vi "Modify Files.vi"() -> ()   [LabVIEW 2015]
uses:
  <vilib>/regexp/Match Regular Expression.xnode
  <userlib>/_OpenG.lib/file/file.llb/Strip Path Extension - String__ogtk.vi
panel:
  out "Array 2":T1(array[cluster])
  out "Array":path[](array[path])
  out "size(s) 2":i32
  out "size(s)":i32
  out "spreadsheet string":string
  # "UFileCrc32"
  # "INPUT: at blockdiagramm"
  # "Look out: some  *.pas files  do  not have a *.dcu file\nwhen included like\n{$I I_Connector_Diff.pas}"
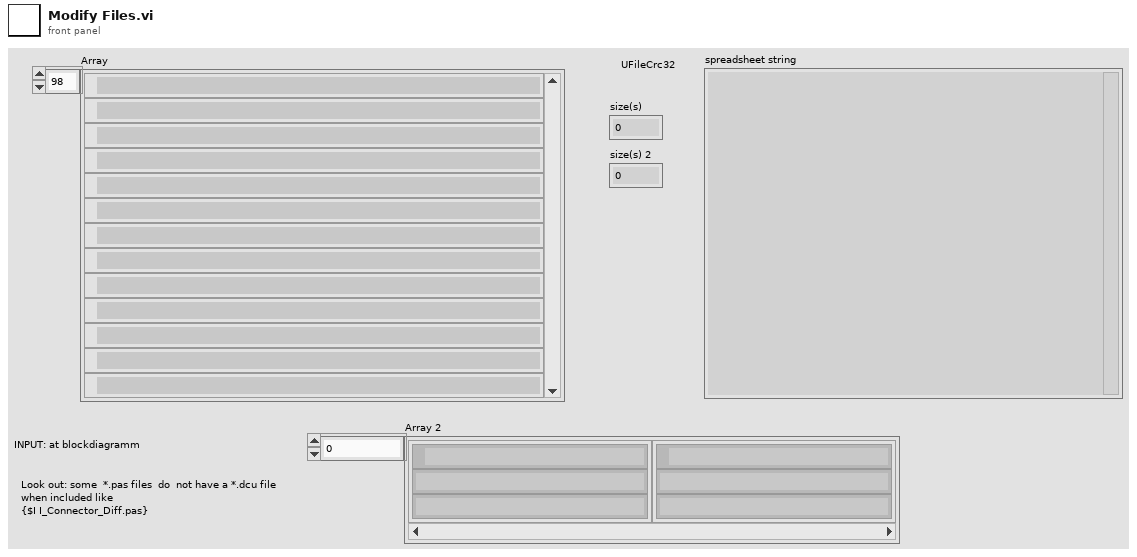
[diagram p1: front panel]
types:
  T1 = cluster{"Path":path, "whole match":string, string}[]
  T2 = enum16{"DebInit add Exit", "Find DebInit", "Find DebFinal", "DebInit with Exit to InitFinal_Add", "uses add InitFinal_List", "add Unit_Name", "InitFinal_Add adapt", "Add InitVars_Dll", "Find Without InitVars_Dll"}
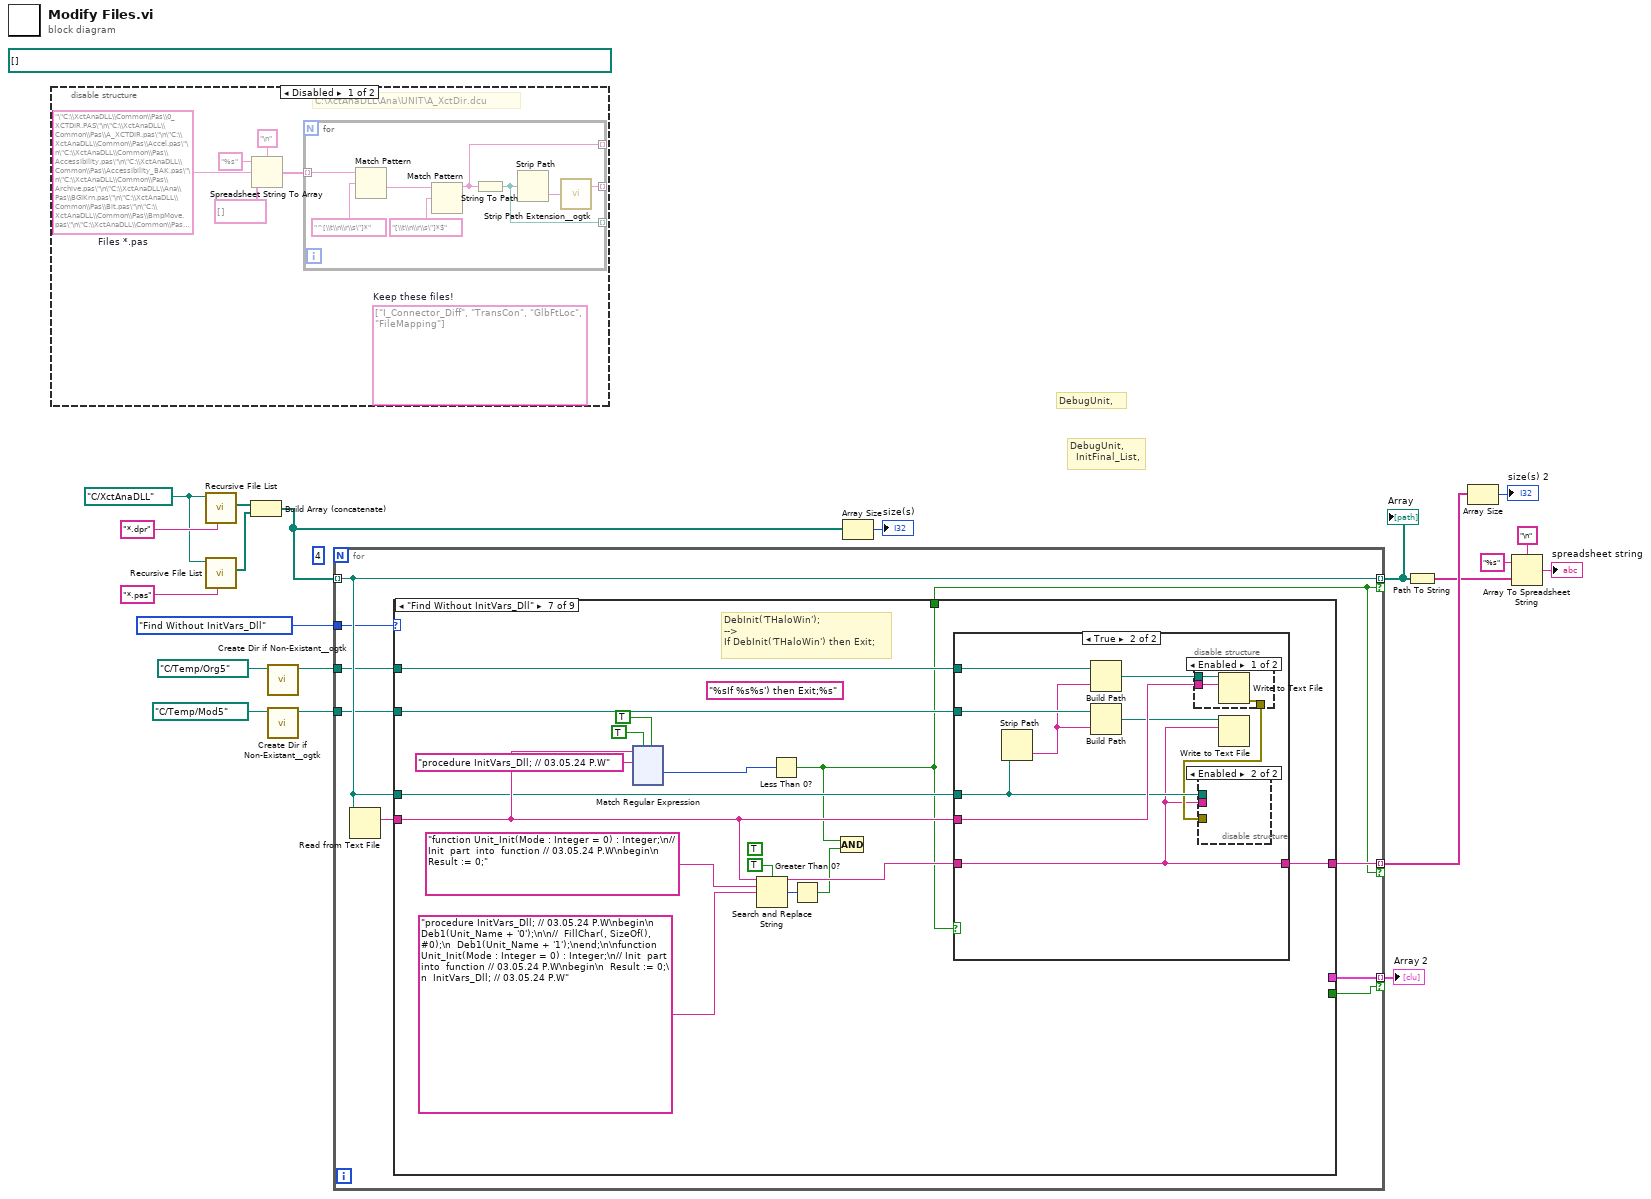
[diagram p0: block diagram]
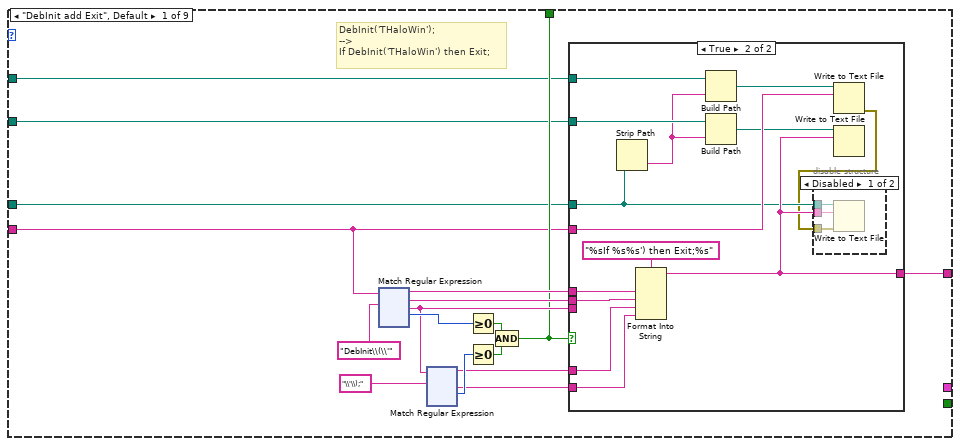
[diagram p3: hidden frame]
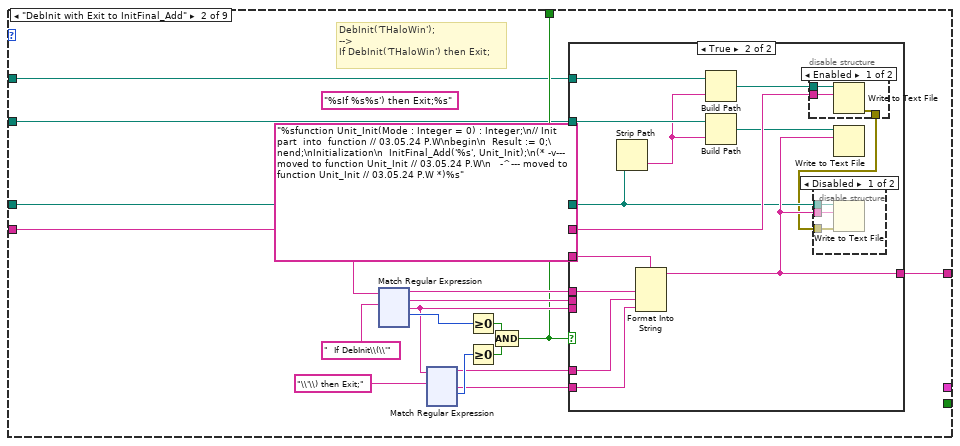
[diagram p6: hidden frame]
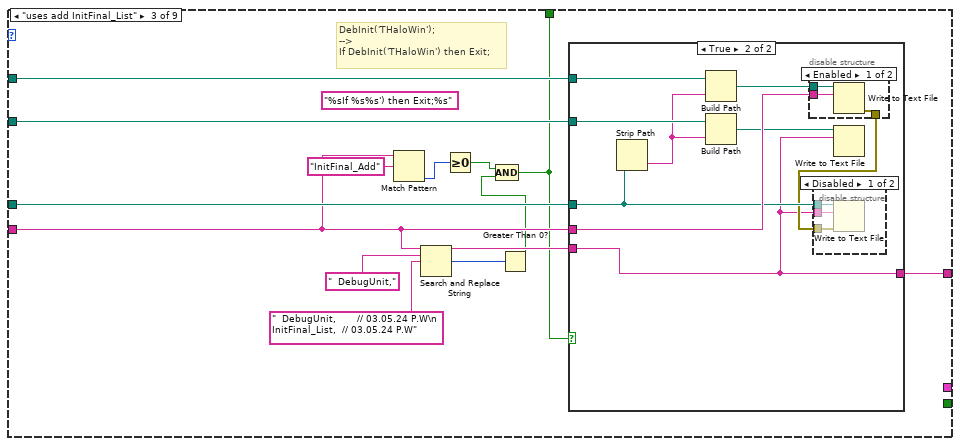
[diagram p10: hidden frame]
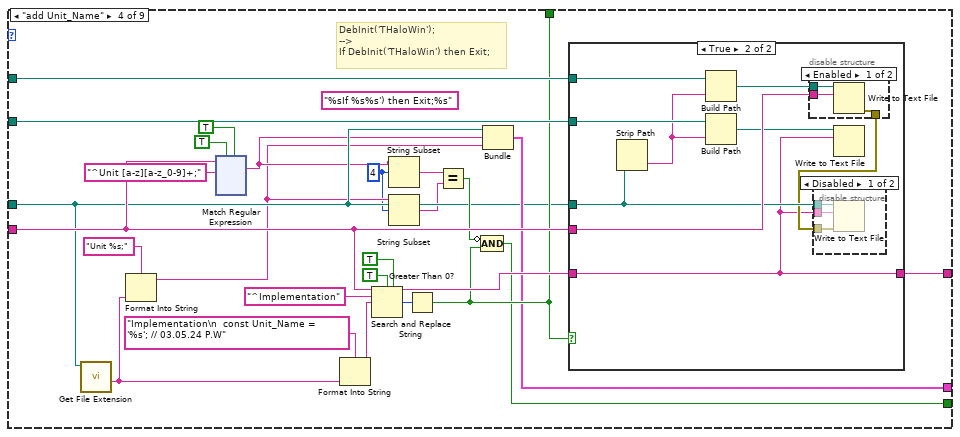
[diagram p14: hidden frame]
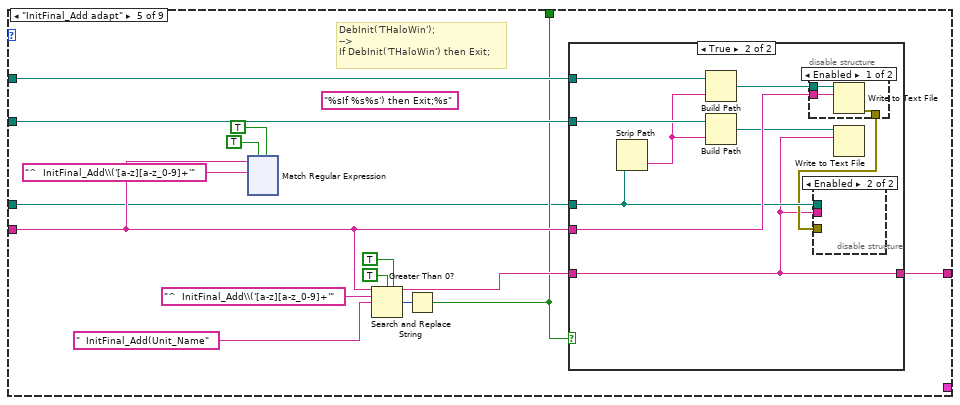
[diagram p18: hidden frame]
diagram:
  (unwired) 4
  w6 = path "C:/XctAnaDLL" ("Folder Path")
  (unwired) path[] []
  # "DebugUnit,\n  InitFinal_List,"
  # "DebugUnit,"
  n1 = disable-structure shown="Disabled" {
    frame Disabled {
      (unwired) string[] ["I_Connector_Diff", "TransCon", "GlbFtLoc", "FileMapping"]  # Keep these files!
      w22 = "\"C:\\XctAnaDLL\\Common\\Pas\\0_XCTDIR.PAS\"\n\"C:\\XctAnaDLL\\Common\\Pas\\A_XCTDIR.pas\"\n\"C:\\XctAnaDLL\\Common\\Pas\\Accel.pas\"\n\"C:\\XctAnaDLL\\Common\\Pas\\Accessibility.pas\"\n\"C:\\XctAnaDLL\\Common\\Pas\\Accessibility_BAK.pas\"\n\"C:\\XctAnaDLL\\Common\\Pas\\Archive.pas\"\n\"C:\\XctAnaDLL\\Ana\\Pas\\BGIKrn.pas\"\n\"C:\\XctAnaDLL\\Common\\Pas\\Bit.pas\"\n\"C:\\XctAnaDLL\\Common\\Pas\\BmpMove.pas\"\n\"C:\\XctAnaDLL\\Common\\Pas\\BmpStack.pas\"\n\"C:\\XctAnaDLL\\Common\\Pas\\BmpUse.pas\"\n\"C:\\XctAnaDLL\\Common\\Pas\\BNHead0.pas\"\n\"C:\\XctAnaDLL\\Ana\\Pas\\BNKEY0.pas\"\n\"C:\\XctAnaDLL\\Ana\\Pas\\BnKnDaKo.pas\"\n\"C:\\XctAnaDLL\\Ana\\Pas\\BNLOCK.pas\"\n\"C:\\XctAnaDLL\\Ana\\Pas\\BufferNumbers.pas\"\n\"C:\\XctAnaDLL\\Ana\\Pas\\BufferNumbers_2.pas\"\n\"C:\\XctAnaDLL\\Ana\\Pas\\Calc.pas\"\n\"C:\\XctAnaDLL\\Common\\Pas\\CheckDat.pas\"\n\"C:\\XctAnaDLL\\Common\\Pas\\CheckPrevious.pas\"\n\"C:\\XctAnaDLL\\Ana\\Pas\\CHK540UP.PAS\"\n\"C:\\XctAnaDLL\\Common\\Pas\\ChkSum.pas\"\n\"C:\\XctAnaDLL\\Ana\\Pas\\ChngSide.pas\"\n\"C:\\XctAnaDLL\\Common\\Pas\\ClientViewXctImagesUnit.pas\"\n\"C:\\XctAnaDLL\\Common\\Pas\\ClipBrdUse.pas\"\n\"C:\\XctAnaDLL\\Ana\\Pas\\cmConst.pas\"\n\"C:\\XctAnaDLL\\Ana\\Pas\\CMDPARAM.PAS\"\n\"C:\\XctAnaDLL\\Common\\Pas\\CodeFind.pas\"\n\"C:\\XctAnaDLL\\Common\\Pas\\ColorDlgUse.pas\"\n\"C:\\XctAnaDLL\\Common\\Pas\\ColorModels.pas\"\n\"C:\\XctAnaDLL\\Common\\Pas\\ColorsPlus.pas\"\n\"C:\\XctAnaDLL\\Info\\TempTest\\COMAC000_Msk.pas\"\n\"C:\\XctAnaDLL\\Info\\TempTest\\COMACFEM_Msk.pas\"\n\"C:\\XctAnaDLL\\Common\\Pas\\ComNames.pas\"\n\"C:\\XctAnaDLL\\Common\\Pas\\ComparePathes.pas\"\n\"C:\\XctAnaDLL\\Common\\Pas\\Complexs.pas\"\n\"C:\\XctAnaDLL\\Ana\\Pas\\CONF.PAS\"\n\"C:\\XctAnaDLL\\Common\\Pas\\ControlsUse.pas\"\n\"C:\\XctAnaDLL\\Common\\Pas\\Crt.pas\"\n\"C:\\XctAnaDLL\\Ana\\Pas\\CSV2PAL.pas\"\n\"C:\\XctAnaDLL\\Ana\\Pas\\csvread.pas\"\n\"C:\\XctAnaDLL\\Ana\\Pas\\CSVSTAT.pas\"\n\"C:\\XctAnaDLL\\Ana\\Pas\\CVDOSTXT.PAS\"\n\"C:\\XctAnaDLL\\Common\\Pas\\DataBaseXct.pas\"\n\"C:\\XctAnaDLL\\Common\\Pas\\DebInit.pas\"\n\"C:\\XctAnaDLL\\Common\\Pas\\DebugForm.pas\"\n\"C:\\XctAnaDLL\\Ana\\Pas\\DefDrvs.pas\"\n\"C:\\XctAnaDLL\\Common\\Pas\\DefHTMLOpts.pas\"\n\"C:\\XctAnaDLL\\Common\\Pas\\DelphiCrt.pas\"\n\"C:\\XctAnaDLL\\Common\\Pas\\DialogsSecure.pas\"\n\"C:\\XctAnaDLL\\Common\\Pas\\DIBTools.pas\"\n\"C:\\XctAnaDLL\\Common\\Pas\\DirTool.pas\"\n\"C:\\XctAnaDLL\\Common\\Pas\\DiskTyp.pas\"\n\"C:\\XctAnaDLL\\Common\\Pas\\DlgDeltaTime.pas\"\n\"C:\\XctAnaDLL\\Ana\\Pas\\Do540up.pas\"\n\"C:\\XctAnaDLL\\Ana\\Pas\\DoModify.pas\"\n\"C:\\XctAnaDLL\\Common\\Pas\\Dos.pas\"\n\"C:\\XctAnaDLL\\Common\\Pas\\DosGlb.pas\"\n\"C:\\XctAnaDLL\\Common\\Pas\\DosTimer.pas\"\n\"C:\\XctAnaDLL\\Common\\Pas\\Draw.pas\"\n\"C:\\XctAnaDLL\\Common\\Pas\\DrawGridDialog.pas\"\n\"C:\\XctAnaDLL\\Ana\\Pas\\DUMMY.PAS\"\n\"C:\\XctAnaDLL\\Common\\Pas\\EE_Param.pas\"\n\"C:\\XctAnaDLL\\Common\\Pas\\EE_Param_RW.pas\"\n\"C:\\XctAnaDLL\\Common\\Pas\\EE_Param_Tools.pas\"\n\"C:\\XctAnaDLL\\Common\\Pas\\ErrConst.pas\"\n\"C:\\XctAnaDLL\\Common\\Pas\\EventLog.pas\"\n\"C:\\XctAnaDLL\\Common\\Pas\\EventLogs.pas\"\n\"C:\\XctAnaDLL\\Ana\\Pas\\ExGraph.pas\"\n\"C:\\XctAnaDLL\\Common\\Pas\\ExitTool.pas\"\n\"C:\\XctAnaDLL\\Ana\\Pas\\EXTPLUS.pas\"\n\"C:\\XctAnaDLL\\Ana\\Pas\\FCOUNT.pas\"\n\"C:\\XctAnaDLL\\Common\\Pas\\FemGlb.pas\"\n\"C:\\XctAnaDLL\\Common\\Pas\\FemurPcForm1.pas\"\n\"C:\\XctAnaDLL\\Common\\Pas\\FFTs.pas\"\n\"C:\\XctAnaDLL\\Delphi\\FileMapping.pas\"\n\"C:\\XctAnaDLL\\Common\\Pas\\FileUtils.pas\"\n\"C:\\XctAnaDLL\\Ana\\Pas\\FindEdge.pas\"\n\"C:\\XctAnaDLL\\Common\\Pas\\FirFilter.pas\"\n\"C:\\XctAnaDLL\\Common\\Pas\\FormatedList.pas\"\n\"C:\\XctAnaDLL\\Common\\Pas\\FormatTools.pas\"\n\"C:\\XctAnaDLL\\Ana\\Pas\\formLoopEdit.pas\"\n\"C:\\XctAnaDLL\\Common\\Pas\\FormMountImage.pas\"\n\"C:\\XctAnaDLL\\Ana\\FormTranslate.pas\"\n\"C:\\XctAnaDLL\\Common\\Pas\\Fourier.pas\"\n\"C:\\XctAnaDLL\\Common\\Pas\\FramePaint.pas\"\n\"C:\\XctAnaDLL\\Common\\Pas\\Frames.pas\"\n\"C:\\XctAnaDLL\\Common\\Pas\\FrameScrolledImage.pas\"\n\"C:\\XctAnaDLL\\Common\\Pas\\FrameScrolledImageTool.pas\"\n\"C:\\XctAnaDLL\\Common\\Pas\\FrameToolRect.pas\"\n\"C:\\XctAnaDLL\\Common\\Pas\\frmBnLockPassWd.pas\"\n\"C:\\XctAnaDLL\\Common\\Pas\\frmHexEdit_U.pas\"\n\"C:\\XctAnaDLL\\Common\\Pas\\frmImage.pas\"\n\"C:\\XctAnaDLL\\Common\\Pas\\frmOptsFilesHyperlink.pas\"\n\"C:\\XctAnaDLL\\Common\\Pas\\FrmXCTAbout.pas\"\n\"C:\\XctAnaDLL\\Common\\Pas\\GdiPlusUse.pas\"\n\"C:\\XctAnaDLL\\Common\\Pas\\GeoTools.pas\"\n\"C:\\XctAnaDLL\\Common\\Pas\\GetMovit.pas\"\n\"C:\\XctAnaDLL\\Common\\Pas\\GetTast.pas\"\n\"C:\\XctAnaDLL\\Common\\Pas\\GIFImage.pas\"\n\"C:\\XctAnaDLL\\Common\\Pas\\Glb.pas\"\n\"C:\\XctAnaDLL\\Common\\Pas\\GlbDecs.pas\"\n\"C:\\XctAnaDLL\\Common\\Pas\\GlbFT.pas\"\n\"C:\\XctAnaDLL\\Ana\\Pas\\GlbFtLoc.Pas\"\n\"C:\\XctAnaDLL\\Common\\Pas\\GlbFtLoc.Pas\"\n\"C:\\XctAnaDLL\\Common\\Pas\\GlbHotKey.pas\"\n\"C:\\XctAnaDLL\\Common\\Pas\\GlbKey.pas\"\n\"C:\\XctAnaDLL\\Common\\Pas\\GlbPath.pas\"\n\"C:\\XctAnaDLL\\Common\\Pas\\Glbtools.pas\"\n\"C:\\XctAnaDLL\\Common\\Pas\\GlbType.pas\"\n\"C:\\XctAnaDLL\\Ana\\Pas\\GoXctDir.pas\"\n\"C:\\XctAnaDLL\\Common\\Pas\\Gr_Crt.pas\"\n\"C:\\XctAnaDLL\\Common\\Pas\\Graph0.pas\"\n\"C:\\XctAnaDLL\\Common\\Pas\\GraphGlb.pas\"\n\"C:\\XctAnaDLL\\Common\\Pas\\GraphicsExt.pas\"\n\"C:\\XctAnaDLL\\Common\\Pas\\GridBasic.pas\"\n\"C:\\XctAnaDLL\\Ana\\Pas\\HelpFile.pas\"\n\"C:\\XctAnaDLL\\Common\\Pas\\I_Connector_Diff.pas\"\n\"C:\\XctAnaDLL\\Common\\Pas\\IfTool.pas\"\n\"C:\\XctAnaDLL\\Common\\Pas\\ImgBuf.pas\"\n\"C:\\XctAnaDLL\\Common\\Pas\\ImgMeasTools.pas\"\n\"C:\\XctAnaDLL\\Common\\Pas\\ImgOverview.pas\"\n\"C:\\XctAnaDLL\\Common\\Pas\\IniFilesUse.pas\"\n\"C:\\XctAnaDLL\\Common\\Pas\\IntChar.pas\"\n\"C:\\XctAnaDLL\\Ana\\Pas\\Intopaz.pas\"\n\"C:\\XctAnaDLL\\Common\\Pas\\IoErr.pas\"\n\"C:\\XctAnaDLL\\Common\\Pas\\IOTools.pas\"\n\"C:\\XctAnaDLL\\Common\\Pas\\JobParameter.pas\"\n\"C:\\XctAnaDLL\\JPEG\\jpeg.pas\"\n\"C:\\XctAnaDLL\\Common\\Pas\\JpgUse.pas\"\n\"C:\\XctAnaDLL\\Common\\Pas\\KeyCodes.pas\"\n\"C:\\XctAnaDLL\\Ana\\Pas\\Keys.pas\"\n\"C:\\XctAnaDLL\\Common\\Pas\\KeyState.pas\"\n\"C:\\XctAnaDLL\\Ana\\Pas\\Kn_Debug.pas\"\n\"C:\\XctAnaDLL\\Ana\\Pas\\KN_Err.pas\"\n\"C:\\XctAnaDLL\\Ana\\Pas\\KN_HLP.pas\"\n\"C:\\XctAnaDLL\\Ana\\Pas\\KN_Intpz.pas\"\n\"C:\\XctAnaDLL\\Ana\\Pas\\Kn_Math.pas\"\n\"C:\\XctAnaDLL\\Ana\\Pas\\KN_MI.pas\"\n\"C:\\XctAnaDLL\\Ana\\Pas\\KN_NCONT.pas\"\n\"C:\\XctAnaDLL\\Ana\\Pas\\Kn_NGlb.pas\"\n\"C:\\XctAnaDLL\\Ana\\Pas\\KN_NSPLI.pas\"\n\"C:\\XctAnaDLL\\Ana\\Pas\\KN_PRINT.pas\"\n\"C:\\XctAnaDLL\\Ana\\Pas\\KN_ROI.pas\"\n\"C:\\XctAnaDLL\\Ana\\Pas\\KN_SetUp.pas\"\n\"C:\\XctAnaDLL\\Ana\\Pas\\Kn_Slc.pas\"\n\"C:\\XctAnaDLL\\Ana\\Pas\\KN_SLC0.pas\"\n\"C:\\XctAnaDLL\\Ana\\Pas\\KN_TOPAZ.pas\"\n\"C:\\XctAnaDLL\\Ana\\Pas\\KNHLP.pas\"\n\"C:\\XctAnaDLL\\Ana\\Pas\\KnMulti.PAS\"\n\"C:\\XctAnaDLL\\Ana\\Pas\\LabViewAna.pas\"\n\"C:\\XctAnaDLL\\Common\\Pas\\License.pas\"\n\"C:\\XctAnaDLL\\Ana\\Pas\\LicensNo.pas\"\n\"C:\\XctAnaDLL\\Ana\\Pas\\LinTick0.pas\"\n\"C:\\XctAnaDLL\\Ana\\Pas\\loopcfg.pas\"\n\"C:\\XctAnaDLL\\Ana\\Pas\\LoopEditIo.pas\"\n\"C:\\XctAnaDLL\\Ana\\Pas\\LPCF_GLB.pas\"\n\"C:\\XctAnaDLL\\Ana\\Pas\\Lpcftool.pas\"\n\"C:\\XctAnaDLL\\Common\\Pas\\Lv_Tools.pas\"\n\"C:\\XctAnaDLL\\Common\\Pas\\Mail.pas\"\n\"C:\\XctAnaDLL\\Common\\Pas\\MathTool.pas\"\n\"C:\\XctAnaDLL\\Common\\Pas\\MathUse.pas\"\n\"C:\\XctAnaDLL\\Ana\\Pas\\MemTools.pas\"\n\"C:\\XctAnaDLL\\Ana\\Pas\\MenuCons.pas\"\n\"C:\\XctAnaDLL\\Common\\Pas\\MenuIds.pas\"\n\"C:\\XctAnaDLL\\Ana\\Pas\\MenuProc.pas\"\n\"C:\\XctAnaDLL\\Ana\\Pas\\MenuTool.pas\"\n\"C:\\XctAnaDLL\\Common\\Pas\\Minimize.pas\"\n\"C:\\XctAnaDLL\\Common\\Pas\\MsgBox.pas\"\n\"C:\\XctAnaDLL\\Ana\\Pas\\MYREN.pas\"\n\"C:\\XctAnaDLL\\Ana\\Pas\\MyValid.pas\"\n\"C:\\XctAnaDLL\\Ana\\Pas\\NETDEBUG.PAS\"\n\"C:\\XctAnaDLL\\Common\\Pas\\NoXctDir.pas\"\n\"C:\\XctAnaDLL\\Common\\Pas\\Objects.pas\"\n\"C:\\XctAnaDLL\\Common\\Pas\\Objects0.pas\"\n\"C:\\XctAnaDLL\\Common\\Pas\\ObjectsP.pas\"\n\"C:\\XctAnaDLL\\Ana\\Pas\\OEMANSI.PAS\"\n\"C:\\XctAnaDLL\\Ana\\Pas\\OLDVER.pas\"\n\"C:\\XctAnaDLL\\Common\\Pas\\OrientDirUse.pas\"\n\"C:\\XctAnaDLL\\Ana\\Pas\\OVERTYP.pas\"\n\"C:\\XctAnaDLL\\Ana\\Pas\\PAL2CSV.pas\"\n\"C:\\XctAnaDLL\\Common\\Pas\\PauseMsg.pas\"\n\"C:\\XctAnaDLL\\Common\\Pas\\PCX.pas\"\n\"C:\\XctAnaDLL\\Ana\\Pas\\Phan_DLG.pas\"\n\"C:\\XctAnaDLL\\Ana\\Pas\\PifTools.pas\"\n\"C:\\XctAnaDLL\\Common\\Pas\\PntMath.pas\"\n\"C:\\XctAnaDLL\\Common\\Pas\\PowerButton.pas\"\n\"C:\\XctAnaDLL\\Common\\Pas\\PowerButton2.pas\"\n\"C:\\XctAnaDLL\\Common\\Pas\\PrinterGlb.pas\"\n\"C:\\XctAnaDLL\\Common\\Pas\\PrintersFpu.pas\"\n\"C:\\XctAnaDLL\\Common\\Pas\\PrintForm.pas\"\n\"C:\\XctAnaDLL\\Common\\Pas\\PrintFormatted.pas\"\n\"C:\\XctAnaDLL\\Common\\Pas\\PrintTable.pas\"\n\"C:\\XctAnaDLL\\Common\\Pas\\PrnFormatedPages.pas\"\n\"C:\\XctAnaDLL\\Common\\Pas\\ProgressBars.pas\"\n\"C:\\XctAnaDLL\\Common\\Pas\\ReadPar.pas\"\n\"C:\\XctAnaDLL\\Common\\Pas\\Rectangles.pas\"\n\"C:\\XctAnaDLL\\Common\\Pas\\RectGlb.pas\"\n\"C:\\XctAnaDLL\\Ana\\Pas\\Resloop.pas\"\n\"C:\\XctAnaDLL\\Common\\Pas\\ResUse.pas\"\n\"C:\\XctAnaDLL\\Ana\\Pas\\rfdbio.pas\"\n\"C:\\XctAnaDLL\\Common\\Pas\\RichEditUse.pas\"\n\"C:\\XctAnaDLL\\Ana\\Pas\\RoiDialog.pas\"\n\"C:\\XctAnaDLL\\Ana\\Pas\\RoiDialogTools.pas\"\n\"C:\\XctAnaDLL\\Ana\\Pas\\RoiMath.pas\"\n\"C:\\XctAnaDLL\\Common\\Pas\\RollImage.pas\"\n\"C:\\XctAnaDLL\\Common\\Pas\\Round1.pas\"\n\"C:\\XctAnaDLL\\Common\\Pas\\SaverDelphi.pas\"\n\"C:\\XctAnaDLL\\Common\\Pas\\ScanIo0.pas\"\n\"C:\\XctAnaDLL\\Ana\\Pas\\ScrConst.pas\"\n\"C:\\XctAnaDLL\\Ana\\Pas\\Search.pas\"\n\"C:\\XctAnaDLL\\Common\\Pas\\SelectForm.pas\"\n\"C:\\XctAnaDLL\\Common\\Pas\\SerialPortThread.pas\"\n\"C:\\XctAnaDLL\\Common\\Pas\\SerialPortXct.pas\"\n\"C:\\XctAnaDLL\\Common\\Pas\\ServerViewXctImagesUnit.pas\"\n\"C:\\XctAnaDLL\\Ana\\Pas\\SetAvDrv.pas\"\n\"C:\\XctAnaDLL\\Common\\Pas\\SetDecimalPoint.pas\"\n\"C:\\XctAnaDLL\\Ana\\Pas\\SETINI.pas\"\n\"C:\\XctAnaDLL\\Common\\Pas\\ShellLink.pas\"\n\"C:\\XctAnaDLL\\Ana\\Pas\\sparcnst.pas\"\n\"C:\\XctAnaDLL\\Common\\Pas\\SpinEditFloat.pas\"\n\"C:\\XctAnaDLL\\Common\\Pas\\Splines.pas\"\n\"C:\\XctAnaDLL\\Common\\Pas\\StartMeasDialogs.pas\"\n\"C:\\XctAnaDLL\\Common\\Pas\\StreamUse.pas\"\n\"C:\\XctAnaDLL\\Common\\Pas\\StrTool.pas\"\n\"C:\\XctAnaDLL\\Common\\Pas\\SysUse.pas\"\n\"C:\\XctAnaDLL\\Ana\\Pas\\T.PAS\"\n\"C:\\XctAnaDLL\\Ana\\Pas\\T2.PAS\"\n\"C:\\XctAnaDLL\\Ana\\Pas\\T3.PAS\"\n\"C:\\XctAnaDLL\\Ana\\Pas\\T22.PAS\"\n\"C:\\XctAnaDLL\\Ana\\Pas\\TAPP.PAS\"\n\"C:\\XctAnaDLL\\Ana\\Pas\\TAPP2.PAS\"\n\"C:\\XctAnaDLL\\Ana\\Pas\\TDrives.pas\"\n\"C:\\XctAnaDLL\\Common\\Pas\\TeeUse.pas\"\n\"C:\\XctAnaDLL\\Ana\\Pas\\TF.PAS\"\n\"C:\\XctAnaDLL\\Ana\\Pas\\THaloEdi.pas\"\n\"C:\\XctAnaDLL\\Ana\\Pas\\THaloWin.pas\"\n\"C:\\XctAnaDLL\\Common\\Pas\\ThreadView.pas\"\n\"C:\\XctAnaDLL\\Common\\Pas\\TKeyApp.pas\"\n\"C:\\XctAnaDLL\\Ana\\Pas\\TLIST.PAS\"\n\"C:\\XctAnaDLL\\Ana\\Pas\\TMathobj.pas\"\n\"C:\\XctAnaDLL\\Ana\\Pas\\TMenuApp.pas\"\n\"C:\\XctAnaDLL\\Ana\\Pas\\TNHTool.pas\"\n\"C:\\XctAnaDLL\\Common\\Pas\\Tools.pas\"\n\"C:\\XctAnaDLL\\Ana\\Pas\\TRANSCON.PAS\"\n\"C:\\XctAnaDLL\\Common\\Pas\\TRANSCON.PAS\"\n\"C:\\XctAnaDLL\\Common\\Pas\\Translate.pas\"\n\"C:\\XctAnaDLL\\Ana\\TranslateData.pas\"\n\"C:\\XctAnaDLL\\Common\\Pas\\TransX.pas\"\n\"C:\\XctAnaDLL\\Common\\Pas\\TstShlObj.pas\"\n\"C:\\XctAnaDLL\\Ana\\Pas\\TT.PAS\"\n\"C:\\XctAnaDLL\\Ana\\Pas\\TTGRAPHS.PAS\"\n\"C:\\XctAnaDLL\\Ana\\Pas\\TTT.PAS\"\n\"C:\\XctAnaDLL\\Common\\Pas\\TurbExt1.pas\"\n\"C:\\XctAnaDLL\\Common\\Pas\\TurboToDelphi.pas\"\n\"C:\\XctAnaDLL\\Ana\\Pas\\tvedit.pas\"\n\"C:\\XctAnaDLL\\Common\\Pas\\Type_s.pas\"\n\"C:\\XctAnaDLL\\Common\\Pas\\TypesUse.pas\"\n\"C:\\XctAnaDLL\\Common\\Pas\\TZBOXES.pas\"\n\"C:\\XctAnaDLL\\Ana\\Pas\\UBNLock.pas\"\n\"C:\\XctAnaDLL\\Common\\Pas\\UBnlockWin.pas\"\n\"C:\\XctAnaDLL\\Common\\Pas\\UFileCRC32.pas\"\n\"C:\\XctAnaDLL\\Common\\Pas\\UfrmClipBoardTools.pas\"\n\"C:\\XctAnaDLL\\Common\\Pas\\UfrmErrBox.pas\"\n\"C:\\XctAnaDLL\\Ana\\Pas\\UfrmRefReport.pas\"\n\"C:\\XctAnaDLL\\Ana\\Pas\\UfrmShowRef.pas\"\n\"C:\\XctAnaDLL\\Ana\\Pas\\UGetKey.pas\"\n\"C:\\XctAnaDLL\\Common\\Pas\\UMsgDelay.pas\"\n\"C:\\XctAnaDLL\\Common\\Pas\\UniDIB.pas\"\n\"C:\\XctAnaDLL\\Info\\TempTest\\Unit1.pas\"\n\"C:\\XctAnaDLL\\Ana\\Pas\\UParUpd.pas\"\n\"C:\\XctAnaDLL\\Ana\\Pas\\UPD51X.pas\"\n\"C:\\XctAnaDLL\\Ana\\Pas\\UPD52X.pas\"\n\"C:\\XctAnaDLL\\Ana\\Pas\\UReadSet.pas\"\n\"C:\\XctAnaDLL\\Common\\Pas\\UseDelphi.pas\"\n\"C:\\XctAnaDLL\\Common\\Pas\\UseDragDrop.pas\"\n\"C:\\XctAnaDLL\\Common\\Pas\\UseGlbHotKeys.pas\"\n\"C:\\XctAnaDLL\\Common\\Pas\\UseList.pas\"\n\"C:\\XctAnaDLL\\Ana\\Pas\\UseUTIP_2.pas\"\n\"C:\\XctAnaDLL\\Ana\\Pas\\UTA_CBD.pas\"\n\"C:\\XctAnaDLL\\Ana\\Pas\\UTANA.pas\"\n\"C:\\XctAnaDLL\\Ana\\Pas\\UTAna1.pas\"\n\"C:\\XctAnaDLL\\Ana\\Pas\\UTAROI.pas\"\n\"C:\\XctAnaDLL\\Ana\\Pas\\UTArray.pas\"\n\"C:\\XctAnaDLL\\Ana\\Pas\\UTBuffer.pas\"\n\"C:\\XctAnaDLL\\Ana\\Pas\\UTBuffer_2.pas\"\n\"C:\\XctAnaDLL\\Ana\\Pas\\UTCOLDLG.pas\"\n\"C:\\XctAnaDLL\\Ana\\Pas\\UTColor.pas\"\n\"C:\\XctAnaDLL\\Ana\\Pas\\UTDBI.pas\"\n\"C:\\XctAnaDLL\\Common\\Pas\\UtFilt0.pas\"\n\"C:\\XctAnaDLL\\Ana\\Pas\\UTFilter.pas\"\n\"C:\\XctAnaDLL\\Common\\Pas\\UTGenOb.pas\"\n\"C:\\XctAnaDLL\\Ana\\Pas\\UTGENROI.pas\"\n\"C:\\XctAnaDLL\\Ana\\Pas\\UTGrpRes.pas\"\n\"C:\\XctAnaDLL\\Common\\Pas\\UtIni.pas\"\n\"C:\\XctAnaDLL\\Ana\\UTINI_Console.pas\"\n\"C:\\XctAnaDLL\\Ana\\Pas\\UTIP.pas\"\n\"C:\\XctAnaDLL\\Ana\\Pas\\UTIP_2.pas\"\n\"C:\\XctAnaDLL\\Ana\\Pas\\UTKnApp.pas\"\n\"C:\\XctAnaDLL\\Ana\\Pas\\UTKNApp0.pas\"\n\"C:\\XctAnaDLL\\Ana\\Pas\\UTKNAPP1.pas\"\n\"C:\\XctAnaDLL\\Ana\\Pas\\UTKNAPP2.pas\"\n\"C:\\XctAnaDLL\\Ana\\Pas\\UtKnPane.pas\"\n\"C:\\XctAnaDLL\\Ana\\Pas\\UTParam.pas\"\n\"C:\\XctAnaDLL\\Ana\\Pas\\UTRef.pas\"\n\"C:\\XctAnaDLL\\Ana\\Pas\\UTRes.pas\"\n\"C:\\XctAnaDLL\\Ana\\Pas\\UTStd.pas\"\n\"C:\\XctAnaDLL\\Ana\\Pas\\UTTABEL.PAS\"\n\"C:\\XctAnaDLL\\Common\\Pas\\UViewErrScr.pas\"\n\"C:\\XctAnaDLL\\Common\\Pas\\VideHook.pas\"\n\"C:\\XctAnaDLL\\Ana\\Pas\\VidLine.pas\"\n\"C:\\XctAnaDLL\\Common\\Pas\\VidLine01.pas\"\n\"C:\\XctAnaDLL\\Common\\Pas\\ViewGrid.pas\"\n\"C:\\XctAnaDLL\\Common\\Pas\\ViewGridUse.pas\"\n\"C:\\XctAnaDLL\\Ana\\Pas\\ViewQLim.pas\"\n\"C:\\XctAnaDLL\\Common\\Pas\\ViewScreens.pas\"\n\"C:\\XctAnaDLL\\Common\\Pas\\ViewXctImages.pas\"\n\"C:\\XctAnaDLL\\Common\\Pas\\ViewXctServerClientGlb.pas\"\n\"C:\\XctAnaDLL\\Info\\TempTest\\WDBIMSK.PAS\"\n\"C:\\XctAnaDLL\\Common\\Pas\\WindowsEx.pas\"\n\"C:\\XctAnaDLL\\Common\\WinFolders.pas\"\n\"C:\\XctAnaDLL\\Common\\Pas\\WinMessagDialog.pas\"\n\"C:\\XctAnaDLL\\Common\\Pas\\WinTmr.pas\"\n\"C:\\XctAnaDLL\\Common\\Pas\\WinTools.pas\"\n\"C:\\XctAnaDLL\\Common\\Pas\\WM_AddMessages.pas\"\n\"C:\\XctAnaDLL\\Common\\Pas\\XbJobSel.pas\"\n\"C:\\XctAnaDLL\\Common\\Pas\\XctChecks.pas\"\n\"C:\\XctAnaDLL\\Common\\Pas\\XctDirFrm.pas\"\n\"C:\\XctAnaDLL\\Common\\Pas\\XctLicense.pas\"\n\"C:\\XctAnaDLL\\Common\\Pas\\XctSetStartPosition.pas\"\n\"C:\\XctAnaDLL\\Common\\Pas\\XctVersion.pas\"\n\"C:\\XctAnaDLL\\Common\\Pas\\XGlb.pas\"\n\"C:\\XctAnaDLL\\Common\\Pas\\XGLB_FB.PAS\"\n\"C:\\XctAnaDLL\\Common\\Pas\\XMeasGrp.pas\"\n\"C:\\XctAnaDLL\\Ana\\Pas\\XSETPAR.pas\"\n\"C:\\XctAnaDLL\\Ana\\Pas\\XSETUP.pas\"\n\"C:\\XctAnaDLL\\Ana\\Pas\\XTRACT.pas\""  # Files *.pas
      # "C:\\XctAnaDLL\\Ana\\UNIT\\A_XctDir.dcu"
      n2 = Spreadsheet String To Array(delimiter (Tab)="\n", format string="%s", spreadsheet string=w22, array type (2D Dbl)=string[] []) -> (array=w21:string[])
      n3 = for {
        tunnel: [w32] -> _ mode=indexing
        tunnel: w21 -> [w28] mode=indexing
        tunnel: [w27] -> _ mode=indexing
        tunnel: [w26] -> _ mode=indexing
        n4 = Match Pattern(string=w28, regular expression="^[\\t\\n\\r\\s\"]*") -> (after substring=w31:string)  [unwired: 1 in, 3 out]
        n5 = Match Pattern(string=w31, regular expression="[\\t\\n\\r\\s\"]*$") -> (before substring=w26:string)  [unwired: 1 in, 3 out]
        n6 = String To Path(string=w26) -> (path=w27:path)
        n7 = Strip Path(path=w27) -> (name=w33:string)  [unwired: 1 out]
        n8 = call-poly <userlib>:"Strip Path Extension__ogtk.vi"("path"=w33) -> ("root"=w32:string)  [unwired: 1 out]
      }
    }
    frame Enabled {
    }
  }
  n9 = call <vilib>:"Recursive File List.vi"("pattern"="*.dpr", "Folder Path"=w6) -> ("All Files in Dir"=w15:path[])  [unwired: 5 in, 4 out]
  n10 = call <vilib>:"Recursive File List.vi"("pattern"="*.pas", "Folder Path"=w6) -> ("All Files in Dir"=w4:path[])  [unwired: 5 in, 4 out]
  n11 = Build Array (concatenate)(w15, w4) -> (w5:path[])
  n12 = call <userlib>:"Create Dir if Non-Existant__ogtk.vi"("Directory Path"=path "C:/Temp/Org5" ("Folder Path")) -> ("dup Directory Path"=w10:path)  [unwired: 8 in, 2 out]
  n13 = call <userlib>:"Create Dir if Non-Existant__ogtk.vi"("Directory Path"=path "C:/Temp/Mod5" ("Folder Path")) -> ("dup Directory Path"=w9:path)  [unwired: 8 in, 2 out]
  n14 = for {
    tunnel: w5 -> [w39] mode=indexing
    tunnel: [w39] -> w16 mode=indexing if=w41
    tunnel: [w42] -> w3 mode=indexing if=w41
    tunnel: w10 -> [w38]
    tunnel: w9 -> [w37]
    tunnel: T2."Find Without InitVars_Dll" -> [w36]
    tunnel: [w35] -> w1 mode=indexing if=w34
    n15 = Read from Text File(file (use dialog)=w39) -> (text=w40:string)  [unwired: 3 in, 3 out]
    n16 = case shown="\"Find Without InitVars_Dll\"" w36 {
      tunnel: [w49 w312 w583 w624 w768 w914 w1059 w1189 w1435] -> w42
      tunnel: [w48 w311 w570 w607 w756 w898 w1044 w1195 w1441] -> w41
      tunnel: w40 -> [w46 w309 w575 w616 w760 w908 w1053 w1193 w1439]
      tunnel: w39 -> [w45 w308 w582 w604 w755 w904 w1049 w1192 w1438]
      tunnel: w38 -> [w44 w307 w581 w623 w767 w913 w1058 w1191 w1437]
      tunnel: w37 -> [w43 w306 w580 w622 w766 w912 w1057 w1190 w1436]
      tunnel: [_ _ _ w606 _ _ _ _ _] -> w34
      tunnel: [_ _ _ w605 _ _ _ _ _] -> w35
      frame "DebInit add Exit", Default {
        # "DebInit('THaloWin');\n-->\nIf DebInit('THaloWin') then Exit;"
        n17 = xnode "Match Regular Expression"("input string"=w46, "regular expression"="DebInit\\(\\'") -> ("before match"=w53:string, "whole match"=w51:string, "after match"=w50:string, "offset past match"=w58:i32)  [unwired: 4 in, 1 out]
        n18 = xnode "Match Regular Expression"("input string"=w50, "regular expression"="\\'\\);") -> ("before match"=w52:string, "after match"=w47:string, "offset past match"=w57:i32)  [unwired: 4 in, 2 out]
        n19 = Greater Or Equal To 0?(x=w58) -> (x >= 0?=w55:bool)
        n20 = Greater Or Equal To 0?(x=w57) -> (x >= 0?=w54:bool)
        n21 = Compound Arithmetic op=AND(w55, w54) -> (w48:bool)
        n22 = case shown="True" w48 {
          tunnel: w53 -> [_ w70]
          tunnel: w52 -> [_ w72]
          tunnel: w51 -> [_ w73]
          tunnel: w50 -> [_ _]
          tunnel: [_ w66] -> w49
          tunnel: w47 -> [_ w71]
          tunnel: w46 -> [_ w67]
          tunnel: w45 -> [_ w65]
          tunnel: w44 -> [_ w69]
          tunnel: w43 -> [_ w68]
          frame False {
          }
          frame True {
            n23 = Strip Path(path=w65) -> (name=w63:string)  [unwired: 1 out]
            n24 = Format Into String(format string="%sIf %s%s') then Exit;%s", w70, w73, w72, w71) -> (resulting string=w66:string)  [unwired: 2 in, 1 out]
            n25 = Build Path(base path=w69, name or relative path=w63) -> (appended path=w62:path)
            n26 = Build Path(base path=w68, name or relative path=w63) -> (appended path=w61:path)
            n27 = Write to Text File(file (use dialog)=w62, text=w67) -> (error out=w60:errorcluster)  [unwired: 2 in, 2 out]
            n28 = disable-structure shown="Disabled" {
              disable-tunnel: w66 -> [w76 _]
              disable-tunnel: w60 -> [w75 _]
              disable-tunnel: w65 -> [w74 _]
              frame Disabled {
                n29 = Write to Text File(file (use dialog)=w74, text=w76, error in=w75) -> ()  [unwired: 1 in, 3 out]
              }
              frame Enabled {
              }
            }
            n30 = Write to Text File(file (use dialog)=w61, text=w66) -> ()  [unwired: 2 in, 3 out]
          }
        }
      }
      frame "DebInit with Exit to InitFinal_Add" {
        (unwired) "%sIf %s%s') then Exit;%s"
        # "DebInit('THaloWin');\n-->\nIf DebInit('THaloWin') then Exit;"
        n31 = xnode "Match Regular Expression"("input string"=w309, "regular expression"="  If DebInit\\(\\'") -> ("before match"=w316:string, "whole match"=w314:string, "after match"=w313:string, "offset past match"=w321:i32)  [unwired: 4 in, 1 out]
        n32 = xnode "Match Regular Expression"("input string"=w313, "regular expression"="\\'\\) then Exit;") -> ("before match"=w315:string, "after match"=w310:string, "offset past match"=w320:i32)  [unwired: 4 in, 2 out]
        n33 = Greater Or Equal To 0?(x=w321) -> (x >= 0?=w318:bool)
        n34 = Greater Or Equal To 0?(x=w320) -> (x >= 0?=w317:bool)
        n35 = Compound Arithmetic op=AND(w318, w317) -> (w311:bool)
        n36 = case shown="True" w311 {
          tunnel: w316 -> [_ w323]
          tunnel: w315 -> [_ w335]
          tunnel: w314 -> [_ _]
          tunnel: w313 -> [_ _]
          tunnel: [_ w330] -> w312
          tunnel: w310 -> [_ w334]
          tunnel: w309 -> [_ w331]
          tunnel: w308 -> [_ w329]
          tunnel: w307 -> [_ w333]
          tunnel: w306 -> [_ w332]
          tunnel: "%sfunction Unit_Init(Mode : Integer = 0) : Integer;\n// Init  part  into  function // 03.05.24 P.W\nbegin\n  Result := 0;\nend;\nInitialization\n  InitFinal_Add('%s', Unit_Init);\n(* -v--- moved to function Unit_Init // 03.05.24 P.W\n   -^--- moved to function Unit_Init // 03.05.24 P.W *)%s" -> [_ w324]
          frame False {
          }
          frame True {
            n37 = Strip Path(path=w329) -> (name=w328:string)  [unwired: 1 out]
            n38 = Format Into String(format string=w324, w323, w335, w334) -> (resulting string=w330:string)  [unwired: 2 in, 1 out]
            n39 = Build Path(base path=w333, name or relative path=w328) -> (appended path=w327:path)
            n40 = Build Path(base path=w332, name or relative path=w328) -> (appended path=w326:path)
            n41 = disable-structure shown="Enabled" {
              disable-tunnel: w331 -> [w338 _]
              disable-tunnel: w327 -> [w337 _]
              disable-tunnel: [w336 _] -> w325
              frame Enabled {
                n42 = Write to Text File(file (use dialog)=w337, text=w338) -> (error out=w336:errorcluster)  [unwired: 2 in, 2 out]
              }
              frame Disabled {
              }
            }
            n43 = disable-structure shown="Disabled" {
              disable-tunnel: w330 -> [w341 _]
              disable-tunnel: w325 -> [w340 _]
              disable-tunnel: w329 -> [w339 _]
              frame Disabled {
                n44 = Write to Text File(file (use dialog)=w339, text=w341, error in=w340) -> ()  [unwired: 1 in, 3 out]
              }
              frame Enabled {
              }
            }
            n45 = Write to Text File(file (use dialog)=w326, text=w330) -> ()  [unwired: 2 in, 3 out]
          }
        }
      }
      frame "uses add InitFinal_List" {
        (unwired) "%sIf %s%s') then Exit;%s"
        # "DebInit('THaloWin');\n-->\nIf DebInit('THaloWin') then Exit;"
        n46 = Match Pattern(string=w575, regular expression="InitFinal_Add") -> (offset past match=w573:i32)  [unwired: 1 in, 3 out]
        n47 = Search and Replace String(input string=w575, search string="  DebugUnit," ("regular expression"), replace string="  DebugUnit,       // 03.05.24 P.W\n  InitFinal_List,  // 03.05.24 P.W" ("regular expression")) -> (result string=w576:string, number of replacements=w577:i32)  [unwired: 5 in, 2 out]
        n48 = Greater Or Equal To 0?(x=w573) -> (x >= 0?=w572:bool)
        n49 = Greater Than 0?(x=w577) -> (x > 0?=w571:bool)
        n50 = Compound Arithmetic op=AND(w572, w571) -> (w570:bool)
        n51 = case shown="True" w570 {
          tunnel: [_ w584] -> w583
          tunnel: w575 -> [_ w590]
          tunnel: w582 -> [_ w589]
          tunnel: w581 -> [_ w592]
          tunnel: w580 -> [_ w591]
          tunnel: w576 -> [_ w584]
          frame False {
          }
          frame True {
            n52 = Strip Path(path=w589) -> (name=w588:string)  [unwired: 1 out]
            n53 = Build Path(base path=w592, name or relative path=w588) -> (appended path=w587:path)
            n54 = Build Path(base path=w591, name or relative path=w588) -> (appended path=w586:path)
            n55 = disable-structure shown="Enabled" {
              disable-tunnel: w590 -> [w595 _]
              disable-tunnel: w587 -> [w594 _]
              disable-tunnel: [w593 _] -> w585
              frame Enabled {
                n56 = Write to Text File(file (use dialog)=w594, text=w595) -> (error out=w593:errorcluster)  [unwired: 2 in, 2 out]
              }
              frame Disabled {
              }
            }
            n57 = disable-structure shown="Disabled" {
              disable-tunnel: w584 -> [w598 _]
              disable-tunnel: w585 -> [w597 _]
              disable-tunnel: w589 -> [w596 _]
              frame Disabled {
                n58 = Write to Text File(file (use dialog)=w596, text=w598, error in=w597) -> ()  [unwired: 1 in, 3 out]
              }
              frame Enabled {
              }
            }
            n59 = Write to Text File(file (use dialog)=w586, text=w584) -> ()  [unwired: 2 in, 3 out]
          }
        }
      }
      frame "add Unit_Name" {
        w600 = 4 ("offset (0)")
        (unwired) "%sIf %s%s') then Exit;%s"
        # "DebInit('THaloWin');\n-->\nIf DebInit('THaloWin') then Exit;"
        n60 = call <vilib>:"Get File Extension.vi"("file"=w604) -> ("filename without extension"=w610:string)  [unwired: 6 in, 4 out]
        n61 = Format Into String(format string="Unit %s;", w610) -> (resulting string=w601:string)  [unwired: 2 in, 1 out]
        n62 = xnode "Match Regular Expression"("input string"=w616, "regular expression"="^Unit [a-z][a-z_0-9]+;", "ignore case? (F)"=TRUE, "multiline? (F)"=TRUE) -> ("whole match"=w603:string)  [unwired: 2 in, 4 out]
        n63 = Format Into String(format string="Implementation\n  const Unit_Name = '%s'; // 03.05.24 P.W" ("regular expression"), w610) -> (resulting string=w611:string)  [unwired: 2 in, 1 out]
        n64 = Search and Replace String(case sensitive?=TRUE ("ignore case? (F)"), multiline?=TRUE ("multiline? (F)"), input string=w616, search string="^Implementation" ("regular expression"), replace string=w611) -> (result string=w619:string, number of replacements=w620:i32)  [unwired: 3 in, 2 out]
        n65 = String Subset(string=w603, offset (0)=w600) -> (substring=w602:string)  [unwired: 1 in]
        n66 = String Subset(string=w601, offset (0)=w600) -> (substring=w599:string)  [unwired: 1 in]
        n67 = Greater Than 0?(x=w620) -> (x > 0?=w607:bool)
        n68 = Equal?(x=w602, y=w599) -> (x = y?=w608:bool)
        n69 = Compound Arithmetic op=AND(invert w608, w607) -> (w606:bool)
        n70 = Bundle(w604, "whole match"=w603, w601) -> (w605:cluster{path, "whole match":string, string})  [unwired: 1 in]
        n71 = case shown="True" w607 {
          tunnel: [_ w739] -> w624
          tunnel: w616 -> [_ w745]
          tunnel: w604 -> [_ w744]
          tunnel: w623 -> [_ w747]
          tunnel: w622 -> [_ w746]
          tunnel: w619 -> [_ w739]
          frame False {
          }
          frame True {
            n72 = Strip Path(path=w744) -> (name=w743:string)  [unwired: 1 out]
            n73 = Build Path(base path=w747, name or relative path=w743) -> (appended path=w742:path)
            n74 = Build Path(base path=w746, name or relative path=w743) -> (appended path=w741:path)
            n75 = disable-structure shown="Enabled" {
              disable-tunnel: w745 -> [w750 _]
              disable-tunnel: w742 -> [w749 _]
              disable-tunnel: [w748 _] -> w740
              frame Enabled {
                n76 = Write to Text File(file (use dialog)=w749, text=w750) -> (error out=w748:errorcluster)  [unwired: 2 in, 2 out]
              }
              frame Disabled {
              }
            }
            n77 = disable-structure shown="Disabled" {
              disable-tunnel: w739 -> [w753 _]
              disable-tunnel: w740 -> [w752 _]
              disable-tunnel: w744 -> [w751 _]
              frame Disabled {
                n78 = Write to Text File(file (use dialog)=w751, text=w753, error in=w752) -> ()  [unwired: 1 in, 3 out]
              }
              frame Enabled {
              }
            }
            n79 = Write to Text File(file (use dialog)=w741, text=w739) -> ()  [unwired: 2 in, 3 out]
          }
        }
      }
      frame "InitFinal_Add adapt" {
        (unwired) "%sIf %s%s') then Exit;%s"
        # "DebInit('THaloWin');\n-->\nIf DebInit('THaloWin') then Exit;"
        n80 = xnode "Match Regular Expression"("input string"=w760, "regular expression"="^  InitFinal_Add\\('[a-z][a-z_0-9]+'", "ignore case? (F)"=TRUE, "multiline? (F)"=TRUE) -> ()  [unwired: 2 in, 5 out]
        n81 = Search and Replace String(case sensitive?=TRUE ("ignore case? (F)"), multiline?=TRUE ("multiline? (F)"), input string=w760, search string="^  InitFinal_Add\\('[a-z][a-z_0-9]+'" ("regular expression"), replace string="  InitFinal_Add(Unit_Name" ("format string")) -> (result string=w763:string, number of replacements=w764:i32)  [unwired: 3 in, 2 out]
        n82 = Greater Than 0?(x=w764) -> (x > 0?=w756:bool)
        n83 = case shown="True" w756 {
          tunnel: [_ w883] -> w768
          tunnel: w760 -> [_ w889]
          tunnel: w755 -> [_ w888]
          tunnel: w767 -> [_ w891]
          tunnel: w766 -> [_ w890]
          tunnel: w763 -> [_ w883]
          frame False {
          }
          frame True {
            n84 = Strip Path(path=w888) -> (name=w887:string)  [unwired: 1 out]
            n85 = Build Path(base path=w891, name or relative path=w887) -> (appended path=w886:path)
            n86 = Build Path(base path=w890, name or relative path=w887) -> (appended path=w885:path)
            n87 = disable-structure shown="Enabled" {
              disable-tunnel: w889 -> [w894 _]
              disable-tunnel: w886 -> [w893 _]
              disable-tunnel: [w892 _] -> w884
              frame Enabled {
                n88 = Write to Text File(file (use dialog)=w893, text=w894) -> (error out=w892:errorcluster)  [unwired: 2 in, 2 out]
              }
              frame Disabled {
              }
            }
            n89 = disable-structure shown="Enabled" {
              disable-tunnel: w883 -> [w897 _]
              disable-tunnel: w884 -> [w896 _]
              disable-tunnel: w888 -> [w895 _]
              frame Disabled {
                n90 = Write to Text File(file (use dialog)=w895, text=w897, error in=w896) -> ()  [unwired: 1 in, 3 out]
              }
              frame Enabled {
              }
            }
            n91 = Write to Text File(file (use dialog)=w885, text=w883) -> ()  [unwired: 2 in, 3 out]
          }
        }
      }
      frame "Add InitVars_Dll" {
        (unwired) TRUE ("multiline? (F)")
        (unwired) "%sIf %s%s') then Exit;%s"
        # "DebInit('THaloWin');\n-->\nIf DebInit('THaloWin') then Exit;"
        n92 = xnode "Match Regular Expression"("input string"=w908, "regular expression"="procedure InitVars_Dll; // 03.05.24 P.W", "ignore case? (F)"=TRUE, "multiline? (F)"=TRUE) -> ("offset past match"=w900:i32)  [unwired: 2 in, 4 out]
        n93 = Search and Replace String(case sensitive?=TRUE ("ignore case? (F)"), input string=w908, search string="function Unit_Init(Mode : Integer = 0) : Integer;\n// Init  part  into  function // 03.05.24 P.W\nbegin\n  Result := 0;", replace string="procedure InitVars_Dll; // 03.05.24 P.W\nbegin\n  Deb1(Unit_Name + '0');\n\n//  FillChar(, SizeOf(), #0);\n  Deb1(Unit_Name + '1');\nend;\n\nfunction Unit_Init(Mode : Integer = 0) : Integer;\n// Init  part  into  function // 03.05.24 P.W\nbegin\n  Result := 0;\n  InitVars_Dll; // 03.05.24 P.W") -> (result string=w910:string, number of replacements=w911:i32)  [unwired: 4 in, 2 out]
        n94 = Less Than 0?(x=w900) -> (x < 0?=w899:bool)
        n95 = Greater Than 0?(x=w911) -> (x > 0?=w901:bool)
        n96 = Compound Arithmetic op=AND(w899, w901) -> (w898:bool)
        n97 = case shown="True" w898 {
          tunnel: [_ w1029] -> w914
          tunnel: w908 -> [_ w1035]
          tunnel: w904 -> [_ w1034]
          tunnel: w913 -> [_ w1037]
          tunnel: w912 -> [_ w1036]
          tunnel: w910 -> [_ w1029]
          frame False {
          }
          frame True {
            n98 = Strip Path(path=w1034) -> (name=w1033:string)  [unwired: 1 out]
            n99 = Build Path(base path=w1037, name or relative path=w1033) -> (appended path=w1032:path)
            n100 = Build Path(base path=w1036, name or relative path=w1033) -> (appended path=w1031:path)
            n101 = disable-structure shown="Enabled" {
              disable-tunnel: w1035 -> [w1040 _]
              disable-tunnel: w1032 -> [w1039 _]
              disable-tunnel: [w1038 _] -> w1030
              frame Enabled {
                n102 = Write to Text File(file (use dialog)=w1039, text=w1040) -> (error out=w1038:errorcluster)  [unwired: 2 in, 2 out]
              }
              frame Disabled {
              }
            }
            n103 = disable-structure shown="Enabled" {
              disable-tunnel: w1029 -> [w1043 _]
              disable-tunnel: w1030 -> [w1042 _]
              disable-tunnel: w1034 -> [w1041 _]
              frame Disabled {
                n104 = Write to Text File(file (use dialog)=w1041, text=w1043, error in=w1042) -> ()  [unwired: 1 in, 3 out]
              }
              frame Enabled {
              }
            }
            n105 = Write to Text File(file (use dialog)=w1031, text=w1029) -> ()  [unwired: 2 in, 3 out]
          }
        }
      }
      frame "Find Without InitVars_Dll" {
        (unwired) TRUE ("multiline? (F)")
        (unwired) "%sIf %s%s') then Exit;%s"
        # "DebInit('THaloWin');\n-->\nIf DebInit('THaloWin') then Exit;"
        n106 = xnode "Match Regular Expression"("input string"=w1053, "regular expression"="procedure InitVars_Dll; // 03.05.24 P.W", "ignore case? (F)"=TRUE, "multiline? (F)"=TRUE) -> ("offset past match"=w1045:i32)  [unwired: 2 in, 4 out]
        n107 = Search and Replace String(case sensitive?=TRUE ("ignore case? (F)"), input string=w1053, search string="function Unit_Init(Mode : Integer = 0) : Integer;\n// Init  part  into  function // 03.05.24 P.W\nbegin\n  Result := 0;", replace string="procedure InitVars_Dll; // 03.05.24 P.W\nbegin\n  Deb1(Unit_Name + '0');\n\n//  FillChar(, SizeOf(), #0);\n  Deb1(Unit_Name + '1');\nend;\n\nfunction Unit_Init(Mode : Integer = 0) : Integer;\n// Init  part  into  function // 03.05.24 P.W\nbegin\n  Result := 0;\n  InitVars_Dll; // 03.05.24 P.W") -> (result string=w1055:string, number of replacements=w1056:i32)  [unwired: 4 in, 2 out]
        n108 = Less Than 0?(x=w1045) -> (x < 0?=w1044:bool)
        n109 = Greater Than 0?(x=w1056) -> (x > 0?=w1046:bool)
        n110 = Compound Arithmetic op=AND(w1044, w1046) -> ()  [unwired: 1 out]
        n111 = case shown="True" w1044 {
          tunnel: [_ w1174] -> w1059
          tunnel: w1053 -> [_ w1180]
          tunnel: w1049 -> [_ w1179]
          tunnel: w1058 -> [_ w1182]
          tunnel: w1057 -> [_ w1181]
          tunnel: w1055 -> [_ w1174]
          frame False {
          }
          frame True {
            n112 = Strip Path(path=w1179) -> (name=w1178:string)  [unwired: 1 out]
            n113 = Build Path(base path=w1182, name or relative path=w1178) -> (appended path=w1177:path)
            n114 = Build Path(base path=w1181, name or relative path=w1178) -> (appended path=w1176:path)
            n115 = disable-structure shown="Enabled" {
              disable-tunnel: w1180 -> [w1185 _]
              disable-tunnel: w1177 -> [w1184 _]
              disable-tunnel: [w1183 _] -> w1175
              frame Enabled {
                n116 = Write to Text File(file (use dialog)=w1184, text=w1185) -> (error out=w1183:errorcluster)  [unwired: 2 in, 2 out]
              }
              frame Disabled {
              }
            }
            n117 = disable-structure shown="Enabled" {
              disable-tunnel: w1174 -> [w1188 _]
              disable-tunnel: w1175 -> [w1187 _]
              disable-tunnel: w1179 -> [w1186 _]
              frame Disabled {
                n118 = Write to Text File(file (use dialog)=w1186, text=w1188, error in=w1187) -> ()  [unwired: 1 in, 3 out]
              }
              frame Enabled {
              }
            }
            n119 = Write to Text File(file (use dialog)=w1176, text=w1174) -> ()  [unwired: 2 in, 3 out]
          }
        }
      }
      frame "Find DebInit" {
        # "If DebInit('THaloWin') then Exit;"
        n120 = xnode "Match Regular Expression"("input string"=w1193, "regular expression"="DebInit\\(\\'") -> ("before match"=w1199:string, "whole match"=w1197:string, "after match"=w1196:string, "offset past match"=w1204:i32)  [unwired: 4 in, 1 out]
        n121 = xnode "Match Regular Expression"("input string"=w1196, "regular expression"="\\'\\) then") -> ("before match"=w1198:string, "after match"=w1194:string, "offset past match"=w1203:i32)  [unwired: 4 in, 2 out]
        n122 = Greater Or Equal To 0?(x=w1204) -> (x >= 0?=w1201:bool)
        n123 = Greater Or Equal To 0?(x=w1203) -> (x >= 0?=w1200:bool)
        n124 = Compound Arithmetic op=AND(w1201, w1200) -> (w1195:bool)
        n125 = case shown="True" w1195 {
          tunnel: w1199 -> [_ _]
          tunnel: w1198 -> [_ w1206]
          tunnel: w1197 -> [_ _]
          tunnel: w1196 -> [_ _]
          tunnel: w1194 -> [_ _]
          tunnel: w1193 -> [_ _]
          tunnel: w1192 -> [_ _]
          tunnel: w1191 -> [_ _]
          tunnel: w1190 -> [_ _]
          tunnel: [_ w1206] -> w1189
          frame False {
          }
          frame True {
          }
        }
      }
      frame "Find DebFinal" {
        # "If DebInit('THaloWin') then Exit;"
        n126 = xnode "Match Regular Expression"("input string"=w1439, "regular expression"="DebFinal\\(\\'") -> ("before match"=w1445:string, "whole match"=w1443:string, "after match"=w1442:string, "offset past match"=w1450:i32)  [unwired: 4 in, 1 out]
        n127 = xnode "Match Regular Expression"("input string"=w1442, "regular expression"="\\'\\) then") -> ("before match"=w1444:string, "after match"=w1440:string, "offset past match"=w1449:i32)  [unwired: 4 in, 2 out]
        n128 = Greater Or Equal To 0?(x=w1450) -> (x >= 0?=w1447:bool)
        n129 = Greater Or Equal To 0?(x=w1449) -> (x >= 0?=w1446:bool)
        n130 = Compound Arithmetic op=AND(w1447, w1446) -> (w1441:bool)
        n131 = case shown="True" w1441 {
          tunnel: w1445 -> [_ _]
          tunnel: w1444 -> [_ w1452]
          tunnel: w1443 -> [_ _]
          tunnel: w1442 -> [_ _]
          tunnel: w1440 -> [_ _]
          tunnel: w1439 -> [_ _]
          tunnel: w1438 -> [_ _]
          tunnel: w1437 -> [_ _]
          tunnel: w1436 -> [_ _]
          tunnel: [_ w1452] -> w1435
          frame False {
          }
          frame True {
          }
        }
      }
    }
  }
  "Array" <- w16
  "Array 2" <- w1
  n132 = Array Size(array=w5) -> (size(s)=→"size(s)":i32)
  n133 = Path To String(path=w16) -> (string=w2:string[])
  n134 = Array Size(array=w3) -> (size(s)=→"size(s) 2":i32)
  n135 = Array To Spreadsheet String(delimiter (Tab)="\n", array=w2, 3:"%s" ("format string")) -> (spreadsheet string=→"spreadsheet string":string)
